vi "Create JSON Schema Header.vi"(8 "error in (no error)":errorcluster, 10 "Description":string, 11 "Title":string) -> (0 "error out":errorcluster, 3 "JSON Schema out":string)   [LabVIEW 2020, in "JSON Schema Generator.lvlib"]
uses:
  JSON Schema Generator.lvlib
  3ef15e4a-16dd-4668-bce3-ec6b426eb69a.vi
  407c657b-ac49-4f70-a0b2-c47d1b969b7f.vi
  <vilib>/JDP Science/JSONtext/Variant to JSON Text.vi
  <vilib>/JDP Science/JSONtext/LVClass Serializer/JSONtext LVClass Serializer.lvclass
  <vilib>/JDP Science/JSONtext/JSONtext.lvlib
panel:
  out "Map Out":map{string, string}(c390)
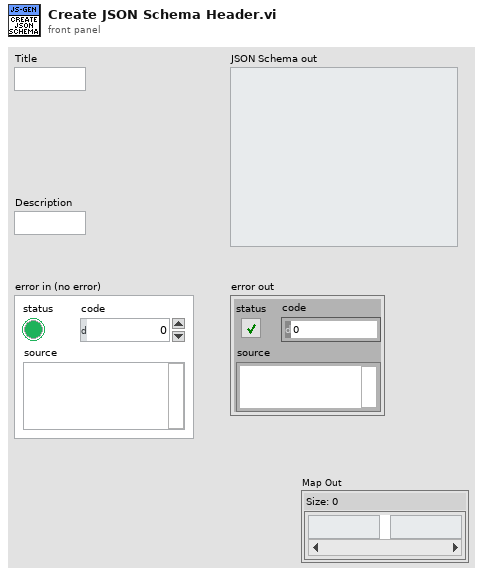
[diagram p1: front panel]
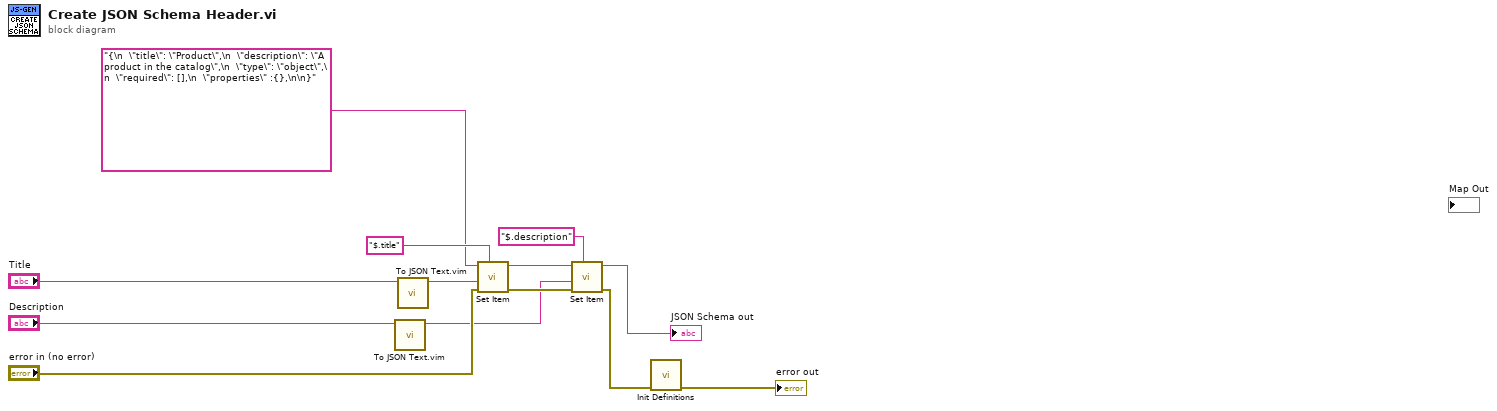
[diagram p0: block diagram]
diagram:
  n1 = call "To JSON Text.vim"("Anything"="Description") -> ("<JSON>"=w3:string)  [unwired: 9 in, 1 out]
  n2 = call "To JSON Text.vim"("Anything"="Title") -> ("<JSON>"=w11:string)  [unwired: 9 in, 1 out]
  n3 = call <vilib>:"Set Item.vi"("$Path or Item Name"="$.title", "error in (no error)"="error in (no error)", "JSON to Insert"=w11, "JSON"="{\n  \"title\": \"Product\",\n  \"description\": \"A product in the catalog\",\n  \"type\": \"object\",\n  \"required\": [],\n  \"properties\" :{},\n\n}") -> ("error out"=w8:errorcluster, "<JSON>"=w6:string)  [unwired: 4 in, 1 out]
  n4 = call <vilib>:"Set Item.vi"("$Path or Item Name"="$.description", "error in (no error)"=w8, "JSON to Insert"=w3, "JSON"=w6) -> ("error out"=w2:errorcluster, "<JSON>"=→"JSON Schema out":string)  [unwired: 4 in, 1 out]
  n5 = call "Init Definitions.vi"("error in (no error)"=w2) -> ("error out (no error)"=→"error out":errorcluster)  [unwired: 10 in]
